vi "4bar Contol Loop.vi"() -> ()   [LabVIEW 2018]
uses:
  <vilib>/Rock Robotics/WPI/ThirdParty/Phoenix-LabVIEW/Motor Controller/Controls/CTRE_Phoenix_MotorControl_NeutralMode.ctl
  Infrastructure/RobotMap.vi
  Infrastructure/Constants.vi
  <vilib>/Rock Robotics/WPI/Switch/WPI_SwitchOpenLimit.vi
  Robot Global Data.vi
  <vilib>/Rock Robotics/WPI/ThirdParty/Phoenix-LabVIEW/Motor Controller/Get/CTRE_Phoenix_MotorController_GetSelectedSensorData.vi
  <vilib>/Rock Robotics/Network Tables/NT Write Number.vi
panel:
  out "4bar Velocity":i32(graph)
  out "4bar Position":i32(graph)
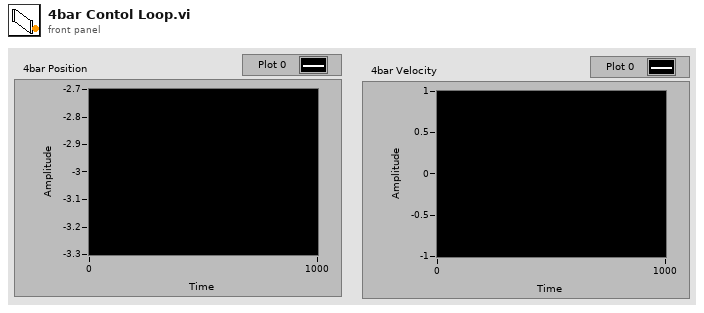
[diagram p1: front panel]
types:
  T1 = typedef "CTRE_Phoenix_MotorControl_NeutralMode.ctl" = enum8{"EEPROMSetting", "Override to Coast", "Override to Brake"}
  T2 = typedef "WPI_MotorControlDeviceRef.ctl" = cluster{"DeviceStatus":errorcluster, "Type":T3, "PWM":cluster{"PWM Channel":T4, "DeadBand":T5}, "CAN":cluster{"Device Number":u8, "SetOutput VI Ref":variant, "GetOutput VI Ref":variant, "Enable VI Ref":variant, "Disable VI Ref":variant, "Data":variant}, "Invert":bool, "DIO PWM":cluster{"PWM \"Enable\" Channel":T4, "DIOChannel":T6, "PWM Rate":dbl}}
  T3 = typedef "WPI_MotorControlType.ctl" = enum16{"PWM", "CAN", "DIO PWM"}
  T4 = typedef "FPGA_DIOPWMChannel.ctl" = enum8{"PWM 0", "PWM 1", "PWM 2", "PWM 3", "PWM 4", "PWM 5", "PWM 6", "PWM 7", "PWM 8", "PWM 9", "PWM MXP 0", "PWM MXP 1", "PWM MXP 2", "PWM MXP 3", "PWM MXP 4", "PWM MXP 5", "PWM MXP 6", "PWM MXP 7", "PWM MXP 8", "PWM MXP 9", "Invalid"}
  T5 = typedef "WPI_PWMDeadband.ctl" = cluster{"Name":string, "maxPositivePwm":i32, "minPositivePwm":i32, "centerPwm":i32, "maxNegativePwm":i32, "minNegativePwm":i32, "angularRange":u16}
  T6 = typedef "FPGA_DIOChannel.ctl" = enum8{"DIO 0", "DIO 1", "DIO 2", "DIO 3", "DIO 4", "DIO 5", "DIO 6", "DIO 7", "DIO 8", "DIO 9", "DIO MXP 0", "DIO MXP 1", "DIO MXP 2", "DIO MXP 3", "DIO MXP 4", "DIO MXP 5", "DIO MXP 6", "DIO MXP 7", "DIO MXP 8", "DIO MXP 9", "DIO MXP 10", "DIO MXP 11", "DIO MXP 12", "DIO MXP 13", "DIO MXP 14", "DIO MXP 15", "SPI Port CS1", "SPI Port CS2", "SPI Port CS3", "SPI Port MISO", "SPI Port MOSI", "Invalid"}
  T7 = typedef "WPI_SwitchDevRef.ctl" = cluster{"DevStatus":errorcluster, "DIO Channel":T6, "CntIndex":T8, "Normally Closed":bool}
  T8 = typedef "FPGA_CounterCtrSystemIndex.ctl" = enum8{"Ctr 0", "Ctr 1", "Ctr 2", "Ctr 3", "Ctr 4", "Ctr 5", "Ctr 6", "Ctr 7", "Invalid"}
  T9 = cluster{"P":dbl, "I":dbl, "D":dbl, "F":dbl, "I Zone":dbl}
  T10 = cluster{"Cruise Velocity":i32, "Acceleration":i32}
  T11 = typedef "CTRE_Phoenix_MotorControl_ControlMode.ctl" = u16
  T12 = cluster{"Control Mode":T11, "Operator Right Joystick Y out":dbl}
  T13 = cluster{"Position (Raw Sensor Units)":i32, "Velocity (Raw Sensor Units per 100 ms)":i32}
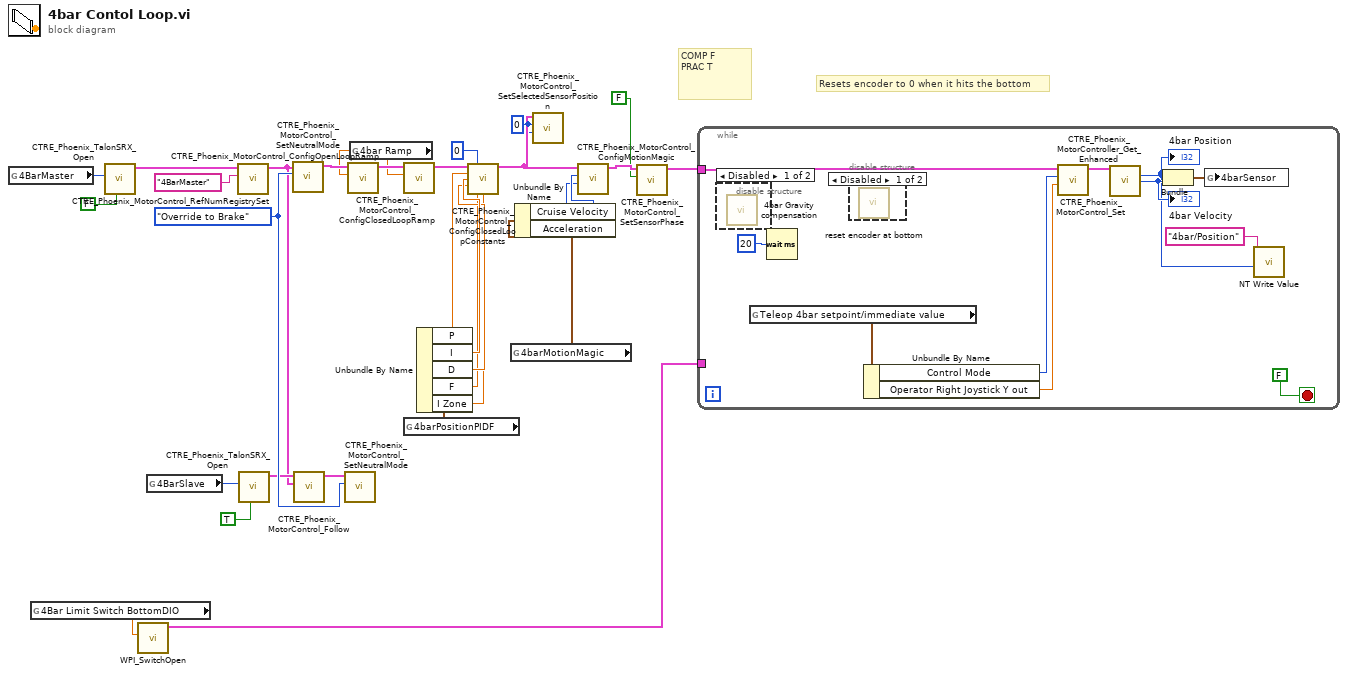
[diagram p0: block diagram]
diagram:
  w4 = 0 ("New Sensor Position")
  w31 = CTRE_Phoenix_MotorControl_NeutralMode."Override to Brake" ("Motor Control Neutral Mode")
  # "COMP F\nPRAC T"
  # "Resets encoder to 0 when it hits the bottom"
  n1 = global read "RobotMap.vi" "4BarMaster"() -> (w23:u8)
  n2 = global read "RobotMap.vi" "4Bar Limit Switch BottomDIO"() -> (w24:dbl)
  n3 = call <vilib>:"CTRE_Phoenix_TalonSRX_Open.vi"("Invert"=FALSE, "Device Number"=w23) -> ("CAN Talon SRX Ref"=w28:T2)  [unwired: 8 in, 1 out]
  n4 = call-poly <vilib>:"WPI_SwitchOpen.vi"("DIO Channel"=w24) -> ("SwitchDevRef"=w25:T7)  [unwired: 9 in, 1 out]
  n5 = global read "RobotMap.vi" "4BarSlave"() -> (w22:u8)
  n6 = call <vilib>:"CTRE_Phoenix_MotorControl_RefNumRegistrySet.vi"("refnum name"="4BarMaster", "PhoenixMotorControlDevRef"=w28) -> ("PhoenixMotorControlDevRef"=w11:T2)  [unwired: 8 in, 1 out]
  n7 = call <vilib>:"CTRE_Phoenix_TalonSRX_Open.vi"("Invert"=TRUE, "Device Number"=w22) -> ("CAN Talon SRX Ref"=w26:T2)  [unwired: 8 in, 1 out]
  n8 = call <vilib>:"CTRE_Phoenix_MotorControl_SetNeutralMode.vi"("Motor Control Neutral Mode"=w31, "PhoenixMotorControlDevRef"=w11) -> ("PhoenixMotorControlDevRef"=w27:T2)  [unwired: 8 in, 1 out]
  n9 = call <vilib>:"CTRE_Phoenix_MotorControl_Follow.vi"("Master Controller to Follow"=w11, "PhoenixMotorControlDevRef"=w26) -> ("PhoenixMotorControlDevRef"=w30:T2)  [unwired: 8 in, 1 out]
  n10 = call <vilib>:"CTRE_Phoenix_MotorControl_SetNeutralMode.vi"("Motor Control Neutral Mode"=w31, "PhoenixMotorControlDevRef"=w30) -> ()  [unwired: 8 in, 2 out]
  n11 = global read "Constants.vi" "4bar Ramp"() -> (w20:dbl)
  n12 = call <vilib>:"CTRE_Phoenix_MotorControl_ConfigOpenLoopRamp.vi"("secondsFromNeutralToFull"=w20, "PhoenixMotorControlDevRef"=w27) -> ("PhoenixMotorControlDevRef"=w21:T2)  [unwired: 8 in, 1 out]
  n13 = call <vilib>:"CTRE_Phoenix_MotorControl_ConfigClosedLoopRamp.vi"("secondsFromNeutralToFull"=w20, "PhoenixMotorControlDevRef"=w21) -> ("PhoenixMotorControlDevRef"=w13:T2)  [unwired: 8 in, 1 out]
  n14 = global read "Constants.vi" "4barPositionPIDF"() -> (w19:T9)
  n15 = Unbundle By Name(w19) -> ("P"=w18:dbl, "I"=w17:dbl, "D"=w16:dbl, "F"=w15:dbl, "I Zone"=w14:dbl)
  n16 = call <vilib>:"CTRE_Phoenix_MotorControl_ConfigClosedLoopConstants.vi"("PhoenixMotorControlDevRef"=w13, "slotIdx"=0, "P"=w18, "I"=w17, "D"=w16, "F"=w15, "I Zone"=w14) -> ("PhoenixMotorControlDevRef"=w5:T2)  [unwired: 7 in, 1 out]
  n17 = global read "Constants.vi" "4barMotionMagic"() -> (w8:T10)
  n18 = Unbundle By Name(w8) -> ("Cruise Velocity"=w7:i32, "Acceleration"=w6:i32)
  n19 = call <vilib>:"CTRE_Phoenix_MotorControl_SetSelectedSensorPosition.vi"("pidLoopIdx"=w4, "New Sensor Position"=w4, "PhoenixMotorControlDevRef"=w5) -> ()  [unwired: 7 in, 2 out]
  n20 = call <vilib>:"CTRE_Phoenix_MotorControl_ConfigMotionMagic.vi"("Acceleration"=w6, "Cruise Velocity"=w7, "PhoenixMotorControlDevRef"=w5) -> ("PhoenixMotorControlDevRef"=w3:T2)  [unwired: 7 in, 1 out]
  n21 = call <vilib>:"CTRE_Phoenix_MotorControl_SetSensorPhase.vi"("PhaseSensor"=FALSE, "PhoenixMotorControlDevRef"=w3) -> ("PhoenixMotorControlDevRef"=w2:T2)  [unwired: 8 in, 1 out]
  n22 = while {
    tunnel: w2 -> [w34]
    tunnel: w25 -> [_]
    stop <- FALSE stop-if-true
    n23 = disable-structure shown="Disabled" {
      frame Disabled {
        n24 = call "4bar Gravity compensation.vi"() -> ()  [unwired: 11 in, 1 out]
      }
      frame Enabled {
      }
    }
    n25 = global read "Robot Global Data.vi" "Teleop 4bar setpoint/immediate value"() -> (w36:T12)
    n26 = Wait (ms)(milliseconds to wait=u32 20) -> ()  [unwired: 1 out]
    n27 = disable-structure shown="Disabled" {
      frame Disabled {
        n28 = call "reset encoder at bottom.vi"() -> ()  [unwired: 11 in, 1 out]
      }
      frame Enabled {
      }
    }
    n29 = Unbundle By Name(w36) -> ("Control Mode"=w40:T11, "Operator Right Joystick Y out"=w37:dbl)
    n30 = call <vilib>:"CTRE_Phoenix_MotorControl_Set.vi"("Output"=w37, "Control Mode"=w40, "PhoenixMotorControlDevRef"=w34) -> ("PhoenixMotorControlDevRef"=w39:T2)  [unwired: 7 in, 1 out]
    n31 = call-poly <vilib>:"CTRE_Phoenix_MotorController_Get_Enhanced.vi"("PhoenixMotorControlDevRef"=w39) -> ("Position (Raw Sensor Units)"=w33:i32, "Velocity (Raw Sensor Units per 100 ms)"=w35:i32)  [unwired: 11 in, 2 out]
    "4bar Position" <- w33
    "4bar Velocity" <- w35
    n32 = Bundle("Position (Raw Sensor Units)"=w33, "Velocity (Raw Sensor Units per 100 ms)"=w35) -> (w38:T13)  [unwired: 1 in]
    n33 = global write "Robot Global Data.vi" "4barSensor"(w38) -> ()
    n34 = call-poly <vilib>:"NT Write Value.vi"("Numeric"=w33, "Name"="4bar/Position") -> ()  [unwired: 9 in, 1 out]
  }
